vi "Report_Name.vi"(8 "error In":errorcluster, 11 "Result":bool=TRUE) -> (0 "error In":errorcluster, 3 "Report Name":string)   [LabVIEW 2021]
panel:
  out "time string":string
  out "date string":string
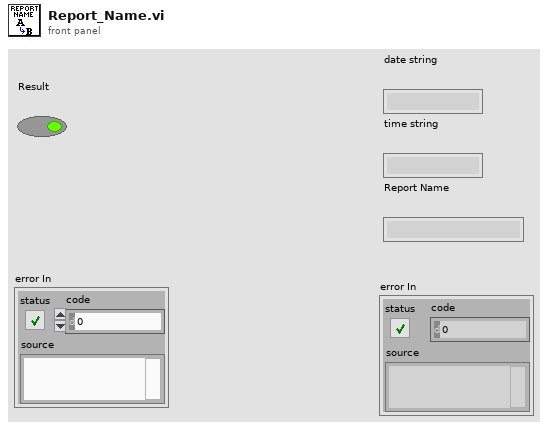
[diagram p1: front panel]
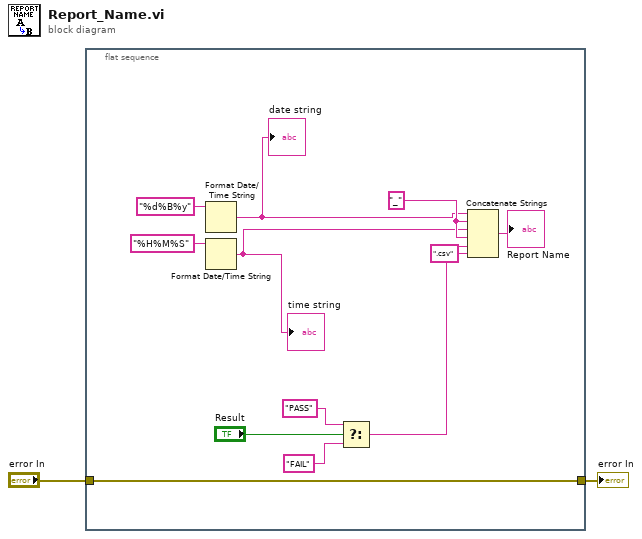
[diagram p0: block diagram]
diagram:
  n1 = flat-sequence {
    tunnel: "error In" -> [w8]
    tunnel: [w8] -> w1
    frame #0 {
      w14 = "_"
      n2 = Format Date/Time String(time format string (%c)="%d%B%y") -> (date/time string=w4:string)  [unwired: 2 in]
      "date string" <- w4
      n3 = Format Date/Time String(time format string (%c)="%H%M%S") -> (date/time string=w3:string)  [unwired: 2 in]
      "time string" <- w3
      n4 = Select(t="PASS", s="Result", f="FAIL") -> (s? t:f=w10:string)
      n5 = Concatenate Strings(w4, w14, w3, w14, w10, ".csv" ("string")) -> (→"Report Name":string)
    }
  }
  "error In" <- w1
